vi "Apply Column Setup After Binding.vi"(7 "DataTable":refnum<class "DataTable.lvclass">, 8 "error in (no error)":errorcluster, 11 "DataGridView in":refnum<class "DataGridView.lvclass">) -> (0 "error out":errorcluster, 3 "DataGridView out":refnum<class "DataGridView.lvclass">)   [LabVIEW 2013, in "DataGrid.lvlib" / "DataGridView.lvclass"]
doc: "This is called after populating the datagridview (via binding its DataTable) so that the custom datatypes can be setup for the columns that require it. This is only needed if you are using <B>Buttons</B> or <B>Combos</B> as all other types are completely automatic."
uses:
  DataGridView.lvclass
  DataTable/DataTable.lvclass
  DataGridView.lvclass/DataGridView.ctl
  System.Windows.Forms
  GridColumn/GridColumn.lvclass/GridColumn.ctl
  GridColumn/GridColumn.lvclass
  GridColumn/Read Params.vi
  GridColumn/Read Caption.vi
  GridColumn/Read Name.vi
  GridColumn/Read AutoSizeMode.vi
  GridColumn/Read FillWeight.vi
  GridColumn/Read datatype.vi
  GridColumn/Read Tooltip.vi
  GridColumn/Read ReadOnly.vi
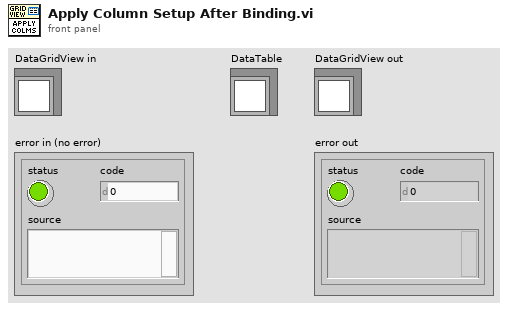
[diagram p1: front panel]
types:
  T1 = typedef "DataGrid.lvlib/GridColumn.lvclass/ColumnType.ctl" = enum16{"string", "image", "check", "numeric", "timestamp", "button", "combo", "link"}
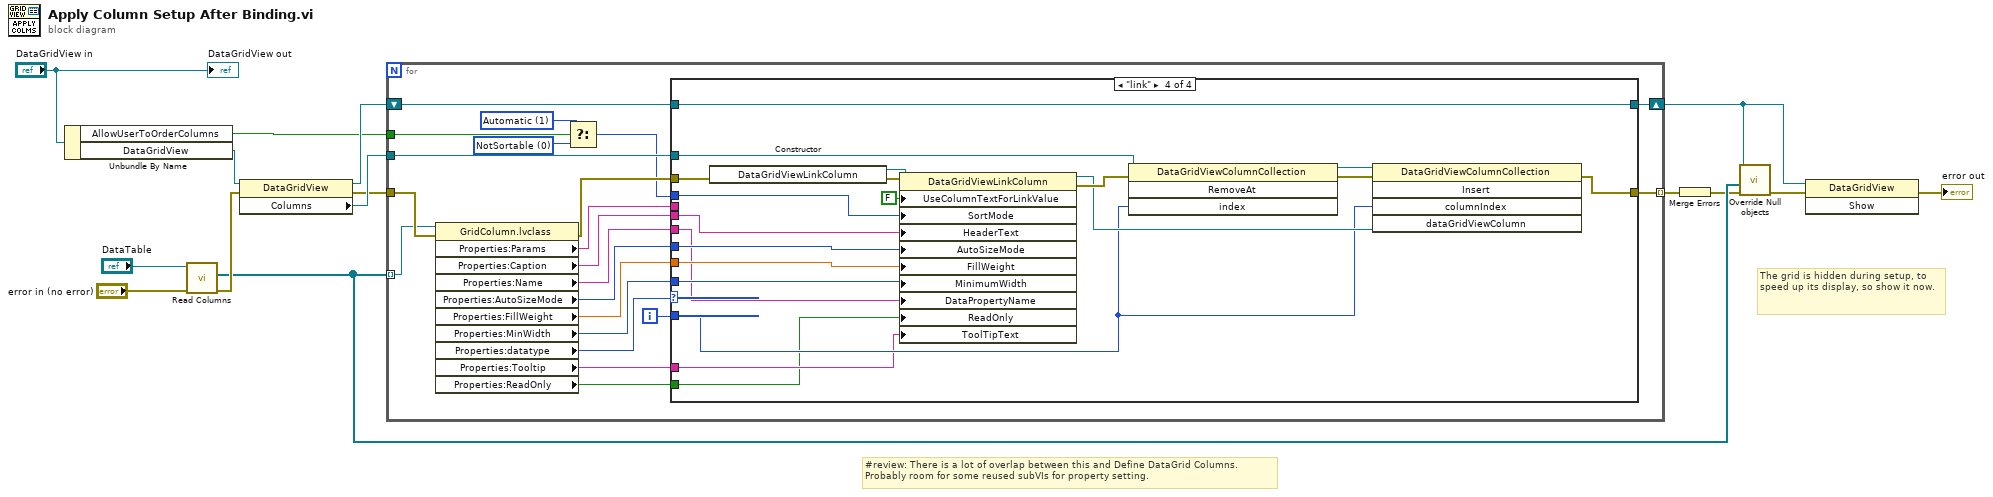
[diagram p0: block diagram]
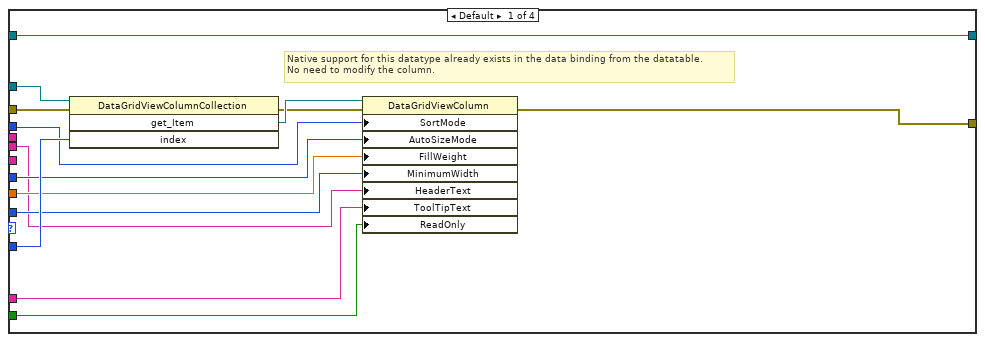
[diagram p2: hidden frame]
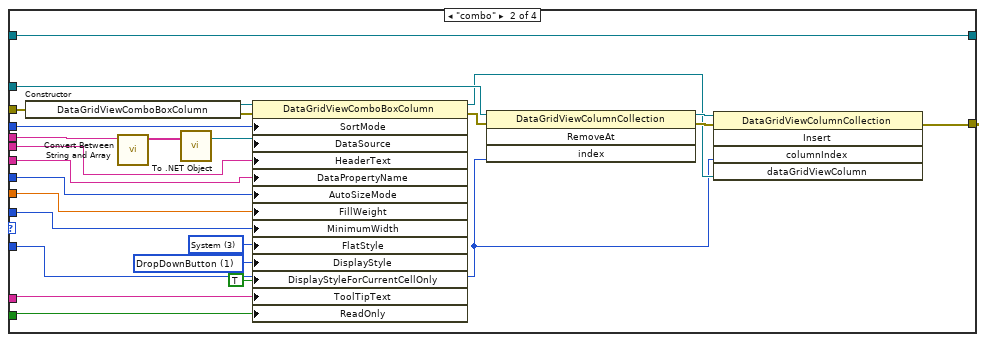
[diagram p3: hidden frame]
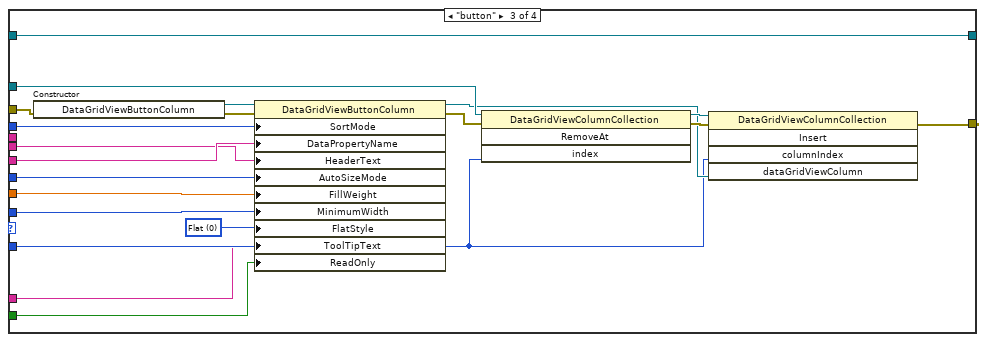
[diagram p4: hidden frame]
diagram:
  # "#review: There is a lot of overlap between this and Define DataGrid Columns. \nProbably room for some reused subVIs for property setting."
  # "The grid is hidden during setup, to speed up its display, so show it now."
  n1 = Unbundle By Name("DataGridView in") -> ("AllowUserToOrderColumns"=w1:bool, "DataGridView"=w13:refnum<k24>)
  n2 = call "Read Columns.vi"("error in (no error)"="error in (no error)", "DataTable in"="DataTable") -> ("error out"=w7:errorcluster, "Columns"=w6:refnum<class "GridColumn.lvclass">[])  [unwired: 7 in, 1 out]
  n3 = property class="DataGridView"(reference=w13, error in=w7) -> (reference out=w3:refnum<k24>, error out=w10:errorcluster, "Columns"=w12:refnum<k24>)
  n4 = for {
    tunnel: w12 -> [w36]
    tunnel: [w35] -> w14 mode=indexing
    tunnel: w10 -> [w26]
    tunnel: w6 -> [w25] mode=indexing
    shift-right: [w22] -> w2
    shift-left: w3 -> [w23]
    tunnel: w1 -> [w19]
    i -> [w34]
    w20 = 1 items=["NotSortable", "Automatic", "Programmatic"] ("SortMode")
    w18 = 0 items=["NotSortable", "Automatic", "Programmatic"] ("SortMode")
    n5 = property class="GridColumn.lvclass"(reference=w25, error in=w26) -> (error out=w27:errorcluster, "Properties:Params"=w33:string, "Properties:Caption"=w24:string, "Properties:Name"=w32:string, "Properties:AutoSizeMode"=w31:i32, "Properties:FillWeight"=w28:sgl, "Properties:MinWidth"=w30:i32, "Properties:datatype"=w29:T1, "Properties:Tooltip"=w21:string, "Properties:ReadOnly"=w16:bool)  [unwired: 1 out]
    n6 = Select(t=w20, s=w19, f=w18) -> (s? t:f=w17:i32)
    n7 = case shown="\"link\"" w29 {
      tunnel: w36 -> [w50 w73 w93 w106]
      tunnel: [w42 w54 w79 w105] -> w35
      tunnel: w34 -> [w49 w55 w80 w99]
      tunnel: w32 -> [_ w60 w85 w102]
      tunnel: w33 -> [_ w63 _ _]
      tunnel: w30 -> [w44 w64 w89 w109]
      tunnel: w28 -> [w45 w65 w88 w110]
      tunnel: w31 -> [w46 w66 w87 w111]
      tunnel: w27 -> [w43 w62 w86 w115]
      tunnel: w24 -> [w41 w61 w84 w101]
      tunnel: w23 -> [w40 w59 w83 w100]
      tunnel: [w40 w59 w83 w100] -> w22
      tunnel: w21 -> [w39 w53 w78 w98]
      tunnel: w17 -> [w38 w52 w77 w97]
      tunnel: w16 -> [w37 w51 w76 w96]
      frame Default {
        # "Native support for this datatype already exists in the data binding from the datatable.\nNo need to modify the column."
        n8 = invoke class="DataGridViewColumnCollection" method="get_Item"(reference=w50, error in=w43, "index"=w49) -> (error out=w47:errorcluster, "get_Item"=w48:refnum<k24>)  [unwired: 1 in, 2 out]
        n9 = property class="DataGridViewColumn"(reference=w48, error in=w47, "SortMode"=w38, "AutoSizeMode"=w46, "FillWeight"=w45, "MinimumWidth"=w44, "HeaderText"=w41, "ToolTipText"=w39, "ReadOnly"=w37) -> (error out=w42:errorcluster)  [unwired: 1 out]
      }
      frame "combo" {
        w57 = 1 items=["ComboBox", "DropDownButton", "Nothing"] ("DisplayStyle")
        w58 = 3 items=["Flat", "Popup", "Standard", "System"] ("FlatStyle")
        n10 = constructor class="DataGridViewComboBoxColumn"(error in=w62) -> (reference out=w75:refnum<k24>, error out=w74:errorcluster)  [unwired: 2 in, 1 out]
        n11 = call "Convert Between String and Array.vi"("String"=w63) -> ("String Array"=w67:string[])  [unwired: 9 in, 1 out]
        n12 = call <vilib>:"To .NET Object.vi"("anything"=w67) -> (".NET object"=w69:refnum<k24>)  [unwired: 1 in, 1 out]
        n13 = property class="DataGridViewComboBoxColumn"(reference=w75, error in=w74, "SortMode"=w52, "DataSource"=w69, "HeaderText"=w61, "DataPropertyName"=w60, "AutoSizeMode"=w66, "FillWeight"=w65, "MinimumWidth"=w64, "FlatStyle"=w58, "DisplayStyle"=w57, "DisplayStyleForCurrentCellOnly"=TRUE, "ToolTipText"=w53, "ReadOnly"=w51) -> (reference out=w70:refnum<k24>, error out=w68:errorcluster)
        n14 = invoke class="DataGridViewColumnCollection" method="RemoveAt"(reference=w73, error in=w68, "index"=w55) -> (reference out=w71:refnum<k24>, error out=w72:errorcluster)  [unwired: 1 in, 2 out]
        n15 = invoke class="DataGridViewColumnCollection" method="Insert"(reference=w71, error in=w72, "columnIndex"=w55, "dataGridViewColumn"=w70) -> (error out=w54:errorcluster)  [unwired: 1 in, 4 out]
      }
      frame "button" {
        w82 = 0 items=["Flat", "Popup", "Standard", "System"] ("FlatStyle")
        n16 = constructor class="DataGridViewButtonColumn"(error in=w86) -> (reference out=w95:refnum<k24>, error out=w94:errorcluster)  [unwired: 2 in, 1 out]
        n17 = property class="DataGridViewButtonColumn"(reference=w95, error in=w94, "SortMode"=w77, "DataPropertyName"=w85, "HeaderText"=w84, "AutoSizeMode"=w87, "FillWeight"=w88, "MinimumWidth"=w89, "FlatStyle"=w82, "ToolTipText"=w78, "ReadOnly"=w76) -> (reference out=w81:refnum<k24>, error out=w90:errorcluster)
        n18 = invoke class="DataGridViewColumnCollection" method="RemoveAt"(reference=w93, error in=w90, "index"=w80) -> (reference out=w91:refnum<k24>, error out=w92:errorcluster)  [unwired: 1 in, 2 out]
        n19 = invoke class="DataGridViewColumnCollection" method="Insert"(reference=w91, error in=w92, "columnIndex"=w80, "dataGridViewColumn"=w81) -> (error out=w79:errorcluster)  [unwired: 1 in, 4 out]
      }
      frame "link" {
        n20 = constructor class="DataGridViewLinkColumn"(error in=w115) -> (reference out=w114:refnum<k24>, error out=w113:errorcluster)  [unwired: 2 in, 1 out]
        n21 = property class="DataGridViewLinkColumn"(reference=w114, error in=w113, "UseColumnTextForLinkValue"=FALSE, "SortMode"=w97, "HeaderText"=w101, "AutoSizeMode"=w111, "FillWeight"=w110, "MinimumWidth"=w109, "DataPropertyName"=w102, "ReadOnly"=w96, "ToolTipText"=w98) -> (reference out=w103:refnum<k24>, error out=w104:errorcluster)
        n22 = invoke class="DataGridViewColumnCollection" method="RemoveAt"(reference=w106, error in=w104, "index"=w99) -> (reference out=w107:refnum<k24>, error out=w108:errorcluster)  [unwired: 1 in, 2 out]
        n23 = invoke class="DataGridViewColumnCollection" method="Insert"(reference=w107, error in=w108, "columnIndex"=w99, "dataGridViewColumn"=w103) -> (error out=w105:errorcluster)  [unwired: 1 in, 4 out]
      }
    }
  }
  n24 = Merge Errors(w14) -> (w5:errorcluster)
  n25 = call "Override Null objects.vi"("error in (no error)"=w5, "Columns"=w6, ".NET Refnum in"=w2) -> ("error out"=w4:errorcluster)  [unwired: 8 in]
  n26 = invoke class="DataGridView" method="Show"(reference=w2, error in=w4) -> (error out=→"error out":errorcluster)  [unwired: 1 in, 2 out]
  "DataGridView out" <- "DataGridView in"
